vi "数据剔除 - WK.vi"(7 "是否启用(T)":bool=TRUE, 8 "错误常量":errorcluster, 9 "是否启用错误(T)":bool=TRUE, 10 "阈值":dbl, 11 "数据输入":dbl) -> (3 "数据输出":dbl)   [LabVIEW 2026, in "UI-温度控制.lvlib" / "Acquisition.lvlib"]
uses:
  Acquisition.lvlib
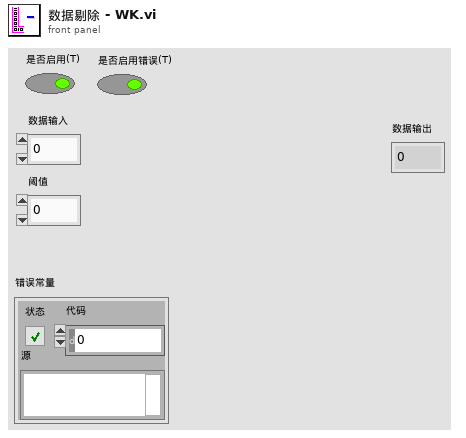
[diagram p1: front panel]
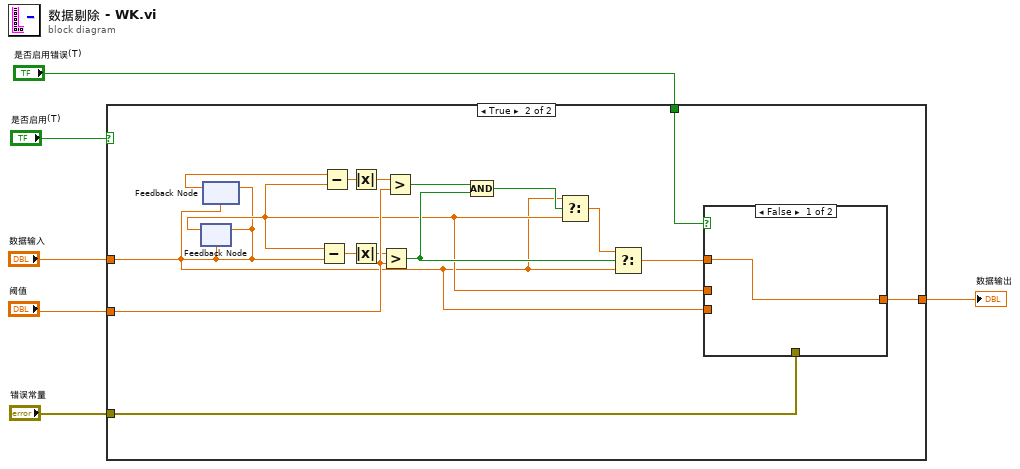
[diagram p0: block diagram]
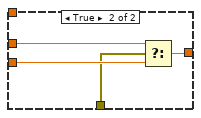
[diagram p3: hidden frame]
diagram:
  n1 = case shown="True" "是否启用(T)" {
    tunnel: "数据输入" -> [w7 w11]
    tunnel: "阈值" -> [_ w23]
    tunnel: [w7 w12] -> w4
    tunnel: "错误常量" -> [_ w9]
    tunnel: "是否启用错误(T)" -> [_ w8]
    frame False {
    }
    frame True {
      n2 = feedback #1(w11) -> (w13:dbl)
      n3 = feedback-in #1(w11) -> ()
      n4 = feedback #2 ("反馈节点")(w11) -> (w18:dbl)
      n5 = feedback-in #2(w11) -> ()
      n6 = Subtract(x=w13, y=w11) -> (x-y=w21:dbl)
      n7 = Subtract(x=w18, y=w13) -> (x-y=w20:dbl)
      n8 = Absolute Value(x=w20) -> (abs(x)=w19:dbl)
      n9 = Absolute Value(x=w21) -> (abs(x)=w22:dbl)
      n10 = Greater?(x=w22, y=w23) -> (0:w16:bool)
      n11 = Greater?(x=w19, y=w23) -> (0:w17:bool)
      n12 = Compound Arithmetic op=AND ("复合运算")(w17, w16) -> (w15:bool)
      n13 = Select(t=w11, s=w15, f=w13) -> (s? t:f=w14:dbl)
      n14 = Select(t=w14, s=w16, f=w11) -> (s? t:f=w10:dbl)
      n15 = case shown="False" w8 {
        tunnel: w13 -> [_ w28]
        tunnel: [w24 w27] -> w12
        tunnel: w11 -> [_ w26]
        tunnel: w10 -> [w24 _]
        tunnel: w9 -> [_ w25]
        frame False {
        }
        frame True {
          n16 = Select(t=w28, s=w25, f=w26) -> (s? t:f=w27:dbl)
        }
      }
    }
  }
  "数据输出" <- w4
